vi "Step_Enter_Phase.vi"(8 "error in (no error)":errorcluster={"status"=FALSE, "code"=0, "source"="\"\""}, 10 "StepContext":string, 11 "Target phase":string) -> (0 "error out":errorcluster={"status"=FALSE, "code"=0, "source"="\"\""}, 2 "status ok":bool, 3 "New StepContext":string)   [LabVIEW 2026]
doc: "INTENT: Centralize phase entry side effects. LOGIC: Record phase start, reset relevant timers and issue required service request once."
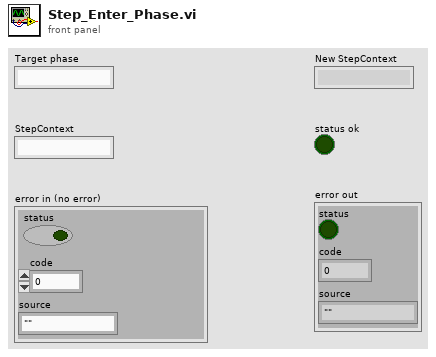
[diagram p1: front panel]
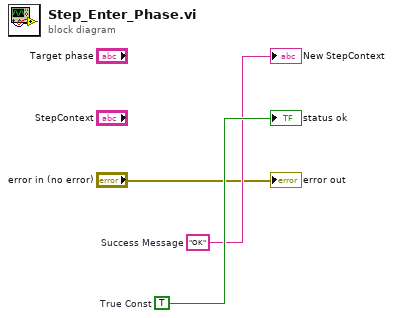
[diagram p0: block diagram]
diagram:
  w3 = TRUE  # True Const
  w2 = "OK"  # Success Message
  "New StepContext" <- w2
  "status ok" <- w3
  "error out" <- "error in (no error)"
